vi "Temps Extra.vi"(6 "x jugador":dbl, 7 "y jugador":dbl, 9 "Temps sense \nmenjar":dbl, 10 "pos y aleatoria":dbl, 11 "pos x aleatoria":dbl) -> (2 "Temps resultant":dbl, 3 "Cluster":cluster{dbl[], dbl[]})   [LabVIEW 2023]
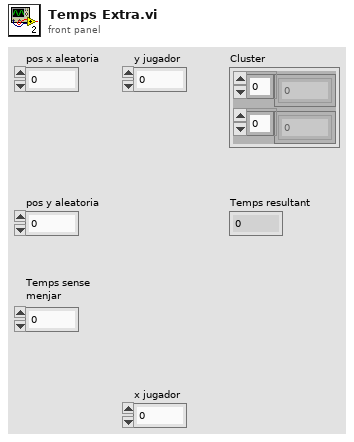
[diagram p1: front panel]
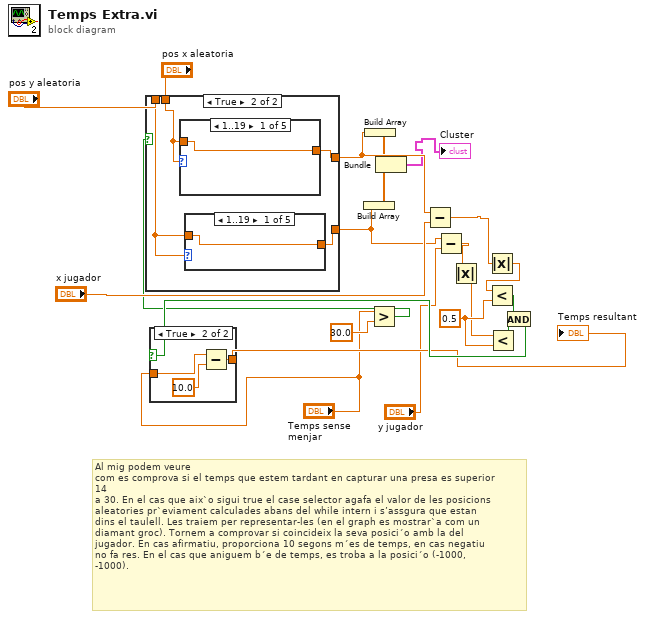
[diagram p0: block diagram]
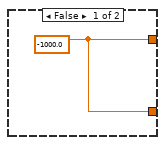
[diagram p3: hidden frame]
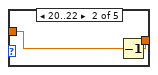
[diagram p4: hidden frame]
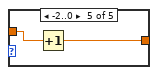
[diagram p7: hidden frame]
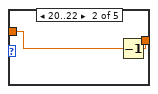
[diagram p8: hidden frame]
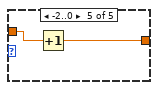
[diagram p11: hidden frame]
diagram:
  w17 = 0.5
  # "Al mig podem veure\ncom es comprova si el temps que estem tardant en capturar una presa es superior\n14\na 30. En el cas que aix`o sigui true el case selector agafa el valor de les posicions\naleatories pr`eviament calculades abans del while intern i s’assgura que estan\ndins el taulell. Les traiem per representar-les (en el graph es mostrar`a com un\ndiamant groc). Tornem a comprovar si coincideix la seva posici´o amb la del\njugador. En cas afirmatiu, proporciona 10 segons m´es de temps, en cas negatiu\nno fa res. En el cas que aniguem b´e de temps, es troba a la posici´o (-1000,\n-1000)."
  n1 = Greater?(x="Temps sense \nmenjar", y=30.0) -> (0:w3:bool)
  n2 = case shown="True" w3 {
    tunnel: [w22 w26] -> w11
    tunnel: [w22 w25] -> w12
    tunnel: "pos y aleatoria" -> [_ w24]
    tunnel: "pos x aleatoria" -> [_ w23]
    frame False {
      w22 = -1000.0
    }
    frame True {
      n3 = case shown="1..19" w23 {
        tunnel: [w34 w36 w37 w38 w40] -> w26
        tunnel: w23 -> [w34 w35 w37 w38 w39]
        frame 1..19 {
        }
        frame 20..22 {
          n4 = Decrement(x=w35) -> (x-1=w36:dbl)
        }
        frame 23.. {
        }
        frame ..-3 {
        }
        frame -2..0 {
          n5 = Increment(x=w39) -> (x+1=w40:dbl)
        }
      }
      n6 = case shown="1..19" w24 {
        tunnel: [w27 w29 w30 w31 w33] -> w25
        tunnel: w24 -> [w27 w28 w30 w31 w32]
        frame 1..19 {
        }
        frame 20..22 {
          n7 = Decrement(x=w28) -> (x-1=w29:dbl)
        }
        frame 23.. {
        }
        frame ..-3 {
        }
        frame -2..0 {
          n8 = Increment(x=w32) -> (x+1=w33:dbl)
        }
      }
    }
  }
  n9 = Build Array(w12) -> (w5:dbl[])
  n10 = Build Array(w11) -> (w4:dbl[])
  n11 = Bundle(w4, w5) -> (→"Cluster":cluster{dbl[], dbl[]})  [unwired: 1 in]
  n12 = Subtract(x=w11, y="x jugador") -> (x-y=w13:dbl)
  n13 = Subtract(x=w12, y="y jugador") -> (x-y=w10:dbl)
  n14 = Absolute Value(x=w10) -> (abs(x)=w8:dbl)
  n15 = Absolute Value(x=w13) -> (abs(x)=w9:dbl)
  n16 = Less?(x=w9, y=w17) -> (x < y?=w6:bool)
  n17 = Less?(x=w8, y=w17) -> (x < y?=w7:bool)
  n18 = And(x=w6, y=w7) -> (x .and. y?=w19:bool)
  n19 = case shown="True" w19 {
    tunnel: "Temps sense \nmenjar" -> [w41 w44]
    tunnel: [w41 w42] -> w16
    frame False {
    }
    frame True {
      n20 = Subtract(x=w44, y=10.0) -> (x-y=w42:dbl)
    }
  }
  "Temps resultant" <- w16
